vi "wait on clock.vi"(8 "error in":errorcluster, 10 "dt":u32=1, 11 "timing source in":refnum<class "ms timing source.lvclass">) -> (0 "error out":errorcluster, 2 "ticks since last call":u32, 3 "timing source out":refnum<class "ms timing source.lvclass">)   [LabVIEW 2013, in "ms timing source.lvclass"]
doc: "This core timing function is used inside of a loop to wait for a clock signal, or dt ticks of a clock signal."
uses:
  ms timing source.lvclass
  ms timing source.lvclass/ms timing source.ctl
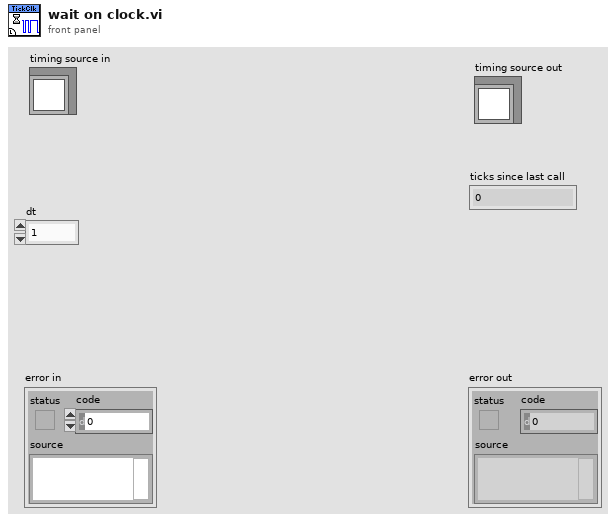
[diagram p1: front panel]
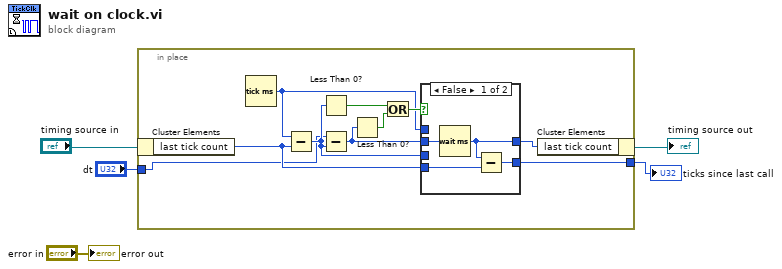
[diagram p0: block diagram]
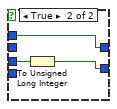
[diagram p2: hidden frame]
diagram:
  n1 = in-place {
    in-place-border: [w11] -> w3
    in-place-border: "dt" -> [w7]
    n2 = in-place-cluster #1("timing source in") -> ("last tick count"=w8:u32)
    n3 = Tick Count (ms)() -> (millisecond timer value=w6:u32)
    n4 = Subtract(x=w6, y=w8) -> (x-y=w10:i64)
    n5 = Less Than 0?(x=w10) -> (x < 0?=w14:bool)
    n6 = Subtract(x=w7, y=w10) -> (x-y=w9:i64)
    n7 = Less Than 0?(x=w9) -> (x < 0?=w15:bool)
    n8 = Or(x=w14, y=w15) -> (x .or. y?=w13:bool)
    n9 = case shown="False" w13 {
      tunnel: [w17 w22] -> w12
      tunnel: w6 -> [_ w22]
      tunnel: [w19 w20] -> w11
      tunnel: w10 -> [_ w21]
      tunnel: w9 -> [w16 _]
      tunnel: w8 -> [w18 _]
      frame False {
        n10 = Wait (ms)(milliseconds to wait=w16) -> (millisecond timer value=w17:u32)
        n11 = Subtract(x=w17, y=w18) -> (x-y=w19:u32)
      }
      frame True {
        n12 = To Unsigned Long Integer(number=w21) -> (unsigned 32bit integer=w20:u32)
      }
    }
    n13 = in-place-cluster #1("last tick count"=w12) -> (→"timing source out":refnum<class "ms timing source.lvclass">)
  }
  "ticks since last call" <- w3
  "error out" <- "error in"
